vi "XYStage.TestLauncher.vi"() -> ()   [LabVIEW 2013]
doc: "JKI State Machine Objects (SMO) 1.0.0.5\nJKI - JKI\nCopyright (c) 2016, JKI"
uses:
  Typedefs/(real)Coords--Cluster.ctl
  Typedefs/(counts)Coords--Cluster.ctl
  XYStage.lvclass
  Typedefs/Configuration--Cluster.ctl
  XYStage.Simulated/XYStage.Simulated.lvclass
  <vilib>/JKI/JKI SMO/SMO/SMO.lvclass/SMO.ctl
  <vilib>/JKI/JKI SMO/SMO/Typedefs/SMOState --Enum.ctl
  <vilib>/JKI/JKI SMO/SMO/Private/ReftoDVR--SMO.vi
  <vilib>/JKI/JKI SMO/SMO/SMO.lvclass
panel:
  in  "Home":bool
  out "Move Complete":bool
  out "Counts":T1
  in  "List Positions":bool
  in  "Move to Position":bool
  in  "Named Positions":i32(listbox)
  in  "Name":string
  in  "Store Position":bool
  out "Current Position":T2
  in  "MoveRel":bool
  in  "Coords":T2
  in  "MoveAbs":bool
  out "error out":errorcluster
  in  "Stop":bool
  # "XY Stage Test Launcher"
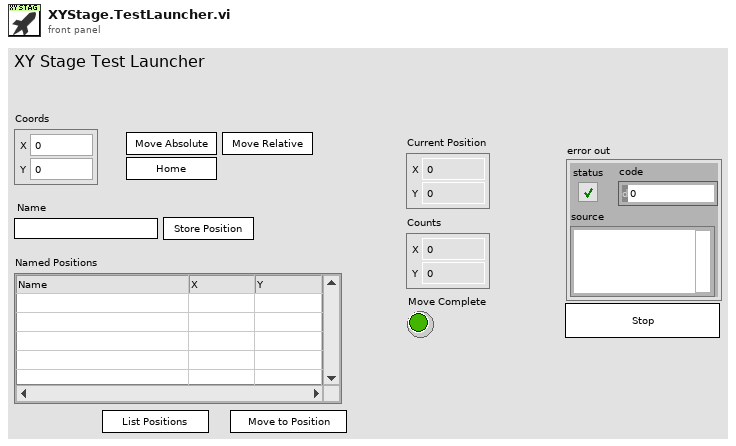
[diagram p1: front panel]
types:
  T1 = typedef "XYStage.lvclass/(counts)Coords--Cluster.ctl" = cluster{"X":i32, "Y":i32}
  T2 = typedef "XYStage.lvclass/(real)Coords--Cluster.ctl" = cluster{"X":dbl, "Y":dbl}
  T3 = typedef "XYStage.lvclass/Configuration--Cluster.ctl" = cluster{"Real-World Units":string, "Counts per Unit":dbl}
  T4 = typedef "SMO.lvclass/Public Events.ctl" = cluster{"Error":refnum<user-event>, "State":refnum<user-event>, "Reserve State":refnum<user-event>}
  T5 = typedef "XYStage.lvclass/PublicEvents--Cluster.ctl" = cluster{"MoveComplete":refnum<user-event>, "NewPosition":refnum<user-event>, "UpdatedNamedPosition":refnum<user-event>, "MoveStarted":refnum<user-event>}
  T6 = cluster{"Event Registration Refnum":refnum<event-registration>}
  T7 = typedef "SMO.lvclass/SMOState --Enum.ctl" = enum16{"unknown", "Created", "Started", "Stopped"}
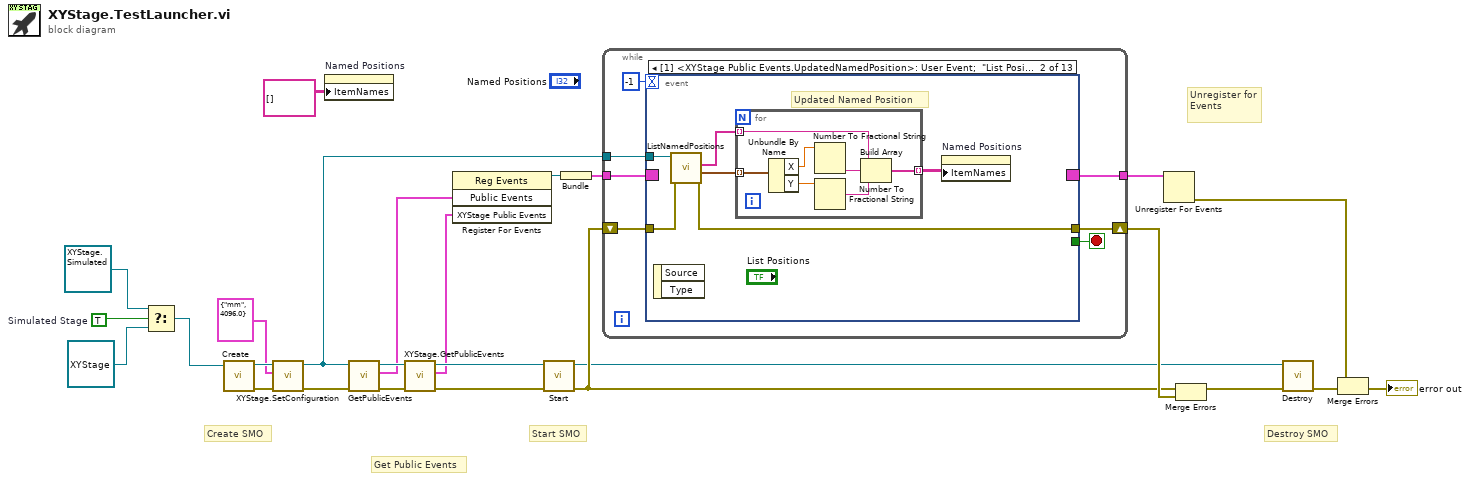
[diagram p0: block diagram]
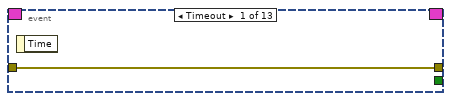
[diagram p2: hidden frame]
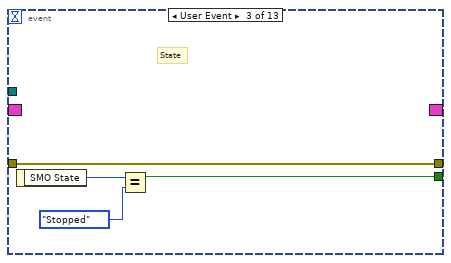
[diagram p3: hidden frame]
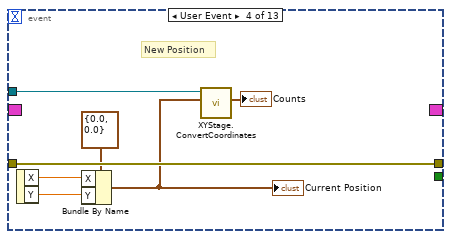
[diagram p4: hidden frame]
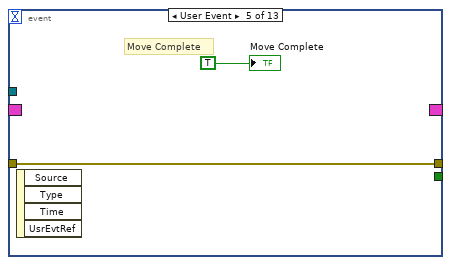
[diagram p5: hidden frame]
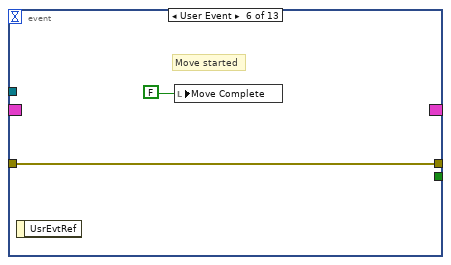
[diagram p6: hidden frame]
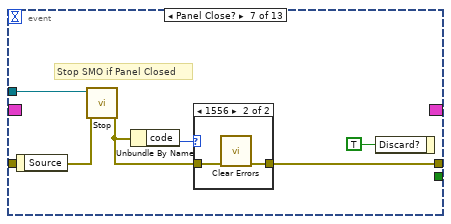
[diagram p7: hidden frame]
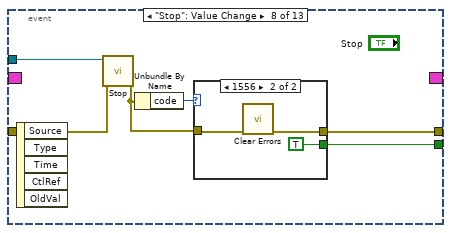
[diagram p9: hidden frame]
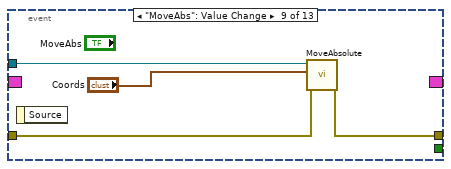
[diagram p11: hidden frame]
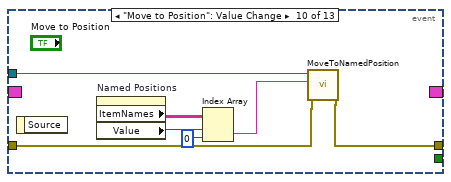
[diagram p12: hidden frame]
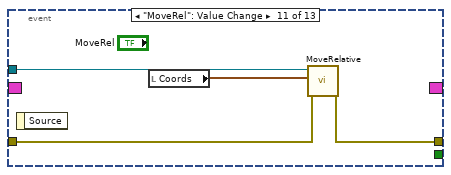
[diagram p13: hidden frame]
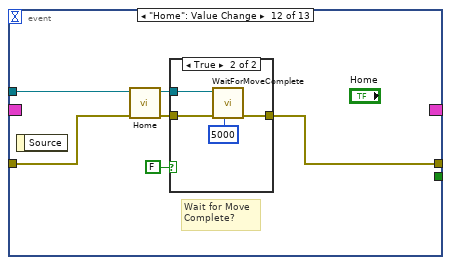
[diagram p14: hidden frame]
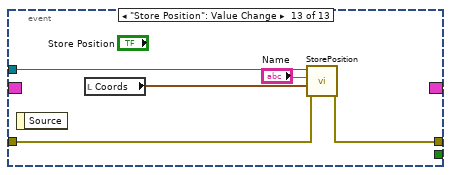
[diagram p16: hidden frame]
diagram:
  w4 = TRUE  # Simulated Stage
  # "Get Public Events"
  # "Start SMO"
  # "Destroy SMO"
  # "Create SMO"
  # "Unregister for Events"
  n1 = Select(t=refnum<class "XYStage.Simulated.lvclass"> refnum ("XYStage.Simulated.lvclass"), s=w4, f=refnum<class "XYStage.lvclass"> refnum ("SMO.Template.lvclass")) -> (s? t:f=w1:refnum<class "XYStage.lvclass">)
  n2 = call <vilib>:"Create.vi"("SMO"=w1) -> ("error out"=w10:errorcluster, "SMO out"=w8:refnum<class "XYStage.lvclass">)  [unwired: 8 in, 1 out]
  n3 = call "XYStage.SetConfiguration.vi"("error in (no error)"=w10, "Configuration"=T3 {"Real-World Units"="mm", "Counts per Unit"=4096.0}, "XYStage"=w8) -> ("error out"=w9:errorcluster, "XYStage out"=w7:refnum<class "XYStage.lvclass">)  [unwired: 7 in]
  n4 = property on="Named Positions" class="MCListbox (strict)"("ItemNames"=string[][] [] ("Item Names")) -> ()  [unwired: 2 in, 2 out]
  n5 = call <vilib>:"GetPublicEvents.vi"("error in (no error)"=w9, "SMO"=w7) -> ("error out"=w12:errorcluster, "Public Events"=w11:T4, "SMO out"=w13:refnum<class "XYStage.lvclass">)  [unwired: 7 in]
  n6 = call "XYStage.GetPublicEvents.vi"("error in (no error)"=w12, "XYStage"=w13) -> ("error out"=w14:errorcluster, "XYStage Public Events"=w16:T5, "XYStage out"=w17:refnum<class "XYStage.lvclass">)  [unwired: 7 in]
  n7 = register-events(w11, w16) -> (reference out=w15:refnum<event-registration>)  [unwired: 2 in, 1 out]
  n8 = call <vilib>:"Start.vi"("error in (no error)"=w14, "SMO"=w17) -> ("error out"=w20:errorcluster, "SMO out"=w18:refnum<class "XYStage.lvclass">)  [unwired: 8 in]
  n9 = Bundle("Event Registration Refnum"=w15) -> (w25:T6)  [unwired: 1 in]
  n10 = while {
    shift-right: [w32] -> w24
    shift-left: w20 -> [w31]
    tunnel: w25 -> [w30]
    tunnel: [w29] -> w26
    tunnel: w7 -> [w28]
    stop <- w33 stop-if-true
    n11 = event shown="[1] <XYStage Public Events.UpdatedNamedPosition>: User Event;  \"List Positions\": Value Change" {
      selector: w30 -> [_ _ _ _ _ _ _ _ _ _ _ _ _]
      dyn-events: [_ _ _ _ _ _ _ _ _ _ _ _ _] -> w29
      timeout: -1 -> [_ _ _ _ _ _ _ _ _ _ _ _ _]
      tunnel: [_ _ w49 _ _ _ _ w72 _ _ _ _ _] -> w33
      tunnel: w28 -> [_ w40 _ w54 _ _ w68 w77 w85 w92 w95 w102 w112]
      tunnel: [w34 w38 w51 w58 w60 w62 w65 w73 w83 w90 w93 w99 w109] -> w32
      tunnel: w31 -> [w34 w39 w51 w58 w60 w62 w67 w76 w84 w91 w94 w98 w110]
      event Timeout {
        n12 = event-data() -> ()  [unwired: 1 in, 1 out]
      }
      event User Event; "List Positions": Value Change {
        # "Updated Named Position"
        n13 = event-data() -> ()  [unwired: 1 in, 2 out]
        n14 = call "ListNamedPositions.vi"("error in (no error)"=w39, "XYStage"=w40) -> ("error out"=w38:errorcluster, "Positions"=w37:T2[], "Names"=w36:string[])  [unwired: 6 in, 1 out]
        n15 = for {
          tunnel: w37 -> [w47] mode=indexing
          tunnel: w36 -> [w44] mode=indexing
          tunnel: [w41] -> w35 mode=indexing
          n16 = Unbundle By Name(w47) -> ("X"=w46:dbl, "Y"=w45:dbl)
          n17 = Number To Fractional String(number=w46) -> (F-format string=w43:string)  [unwired: 3 in]
          n18 = Number To Fractional String(number=w45) -> (F-format string=w42:string)  [unwired: 3 in]
          n19 = Build Array(w44, w43, w42) -> (w41:string[])
        }
        n20 = property on="Named Positions" class="MCListbox (strict)"("ItemNames"=w35) -> ()  [unwired: 2 in, 2 out]
      }
      event User Event {
        # "State"
        n21 = event-data() -> ("SMO State"=w50:T7)  [unwired: 1 in]
        n22 = Equal?(x=w50, y=SMOState_--Enum."Stopped") -> (x = y?=w49:bool)
      }
      event User Event {
        # "New Position"
        n23 = event-data() -> ("X"=w56:dbl, "Y"=w55:dbl)  [unwired: 1 in]
        n24 = Bundle By Name(cluster=T2 {"X"=0.0, "Y"=0.0} ("Coords"), "X"=w56, "Y"=w55) -> (w53:T2)
        "Current Position" <- w53
        n25 = call-dynamic "XYStage.ConvertCoordinates.vi"("Real Units Coords"=w53, "XYStage in"=w54) -> ("Counts out"=→"Counts":T1)  [unwired: 6 in, 3 out]
      }
      event User Event {
        # "Move Complete"
        n26 = event-data() -> ()  [unwired: 1 in, 4 out]
        "Move Complete" <- TRUE
      }
      event User Event {
        # "Move started"
        n27 = event-data() -> ()  [unwired: 1 in, 1 out]
        n28 = local write "Move Complete"(FALSE) -> ()
      }
      event Panel Close? {
        # "Stop SMO if Panel Closed"
        n29 = event-data() -> ()  [unwired: 1 in, 1 out]
        n30 = call <vilib>:"Stop.vi"("error in (no error)"=w67, "SMO"=w68) -> ("error out"=w64:errorcluster)  [unwired: 8 in, 1 out]
        n31 = Unbundle By Name(w64) -> ("code"=w63:i32)
        n32 = case shown="1556" w63 {
          tunnel: w64 -> [w69 w71]
          tunnel: [w69 w70] -> w65
          frame Default {
          }
          frame 1556 {
            n33 = call <vilib>:"Clear Errors.vi"("error in (no error)"=w71) -> ("error out"=w70:errorcluster)  [unwired: 6 in]
          }
        }
        n34 = event-data("Discard?"=TRUE ("OK")) -> ()  [unwired: 1 in, 1 out]
      }
      event "Stop": Value Change {
        n35 = event-data() -> ()  [unwired: 1 in, 5 out]
        n36 = call <vilib>:"Stop.vi"("error in (no error)"=w76, "SMO"=w77) -> ("error out"=w74:errorcluster)  [unwired: 8 in, 1 out]
        n37 = Unbundle By Name(w74) -> ("code"=w75:i32)
        n38 = case shown="1556" w75 {
          tunnel: w74 -> [w78 w81]
          tunnel: [w78 w80] -> w73
          tunnel: [_ TRUE] -> w72
          frame Default {
          }
          frame 1556 {
            n39 = call <vilib>:"Clear Errors.vi"("error in (no error)"=w81) -> ("error out"=w80:errorcluster)  [unwired: 6 in]
          }
        }
      }
      event "MoveAbs": Value Change {
        n40 = event-data() -> ()  [unwired: 1 in, 1 out]
        n41 = call "MoveAbsolute.vi"("error in (no error)"=w84, "Units"="Coords", "XYStage"=w85) -> ("error out"=w83:errorcluster)  [unwired: 7 in, 1 out]
      }
      event "Move to Position": Value Change {
        n42 = event-data() -> ()  [unwired: 1 in, 1 out]
        n43 = property on="Named Positions" class="MCListbox (strict)"() -> ("ItemNames"=w89:string[][], "Value"=w88:i32)  [unwired: 2 in, 2 out]
        n44 = Index Array(array=w89, index (row)=w88, index (col)=0 ("disabled index (col)")) -> (element=w86:string)
        n45 = call "MoveToNamedPosition.vi"("error in (no error)"=w91, "MoveToNamedPosition"=w86, "XYStage"=w92) -> ("error out"=w90:errorcluster)  [unwired: 7 in, 1 out]
      }
      event "MoveRel": Value Change {
        n46 = event-data() -> ()  [unwired: 1 in, 1 out]
        n47 = local read "Coords"() -> (w96:T2)
        n48 = call "MoveRelative.vi"("error in (no error)"=w94, "Units"=w96, "XYStage"=w95) -> ("error out"=w93:errorcluster)  [unwired: 7 in, 1 out]
      }
      event "Home": Value Change {
        # "Wait for Move\nComplete?"
        n49 = event-data() -> ()  [unwired: 1 in, 1 out]
        n50 = call "Home.vi"("error in (no error)"=w98, "XYStage"=w102) -> ("error out"=w100:errorcluster, "XYStage out"=w101:refnum<class "XYStage.lvclass">)  [unwired: 8 in]
        n51 = case shown="True" FALSE {
          tunnel: w101 -> [_ w107]
          tunnel: w100 -> [w103 w106]
          tunnel: [w103 w105] -> w99
          frame False {
          }
          frame True {
            n52 = call "WaitForMoveComplete.vi"("timeout (5000 ms)"=5000, "error in (no error)"=w106, "XYStage"=w107) -> ("error out"=w105:errorcluster)  [unwired: 6 in, 2 out]
          }
        }
      }
      event "Store Position": Value Change {
        n53 = event-data() -> ()  [unwired: 1 in, 1 out]
        n54 = local read "Coords"() -> (w111:T2)
        n55 = call "StorePosition.vi"("error in (no error)"=w110, "Units"=w111, "Name"="Name", "XYStage"=w112) -> ("error out"=w109:errorcluster)  [unwired: 6 in, 1 out]
      }
    }
  }
  n56 = Unregister For Events(event registration refnum=w26) -> (error out=w23:errorcluster)  [unwired: 1 in]
  n57 = Merge Errors(w20, w24) -> (w19:errorcluster)
  n58 = call <vilib>:"Destroy.vi"("error in (no error)"=w19, "SMO"=w18) -> ("error out"=w21:errorcluster)  [unwired: 9 in]
  n59 = Merge Errors(w23, w21) -> (→"error out":errorcluster)
